vi "Add Error.vi"(8 "error in (no error)":errorcluster, 9 "String to Append":string, 10 "Error":T1, 11 "Insert Error":bool=TRUE) -> (0 "error out":errorcluster)   [LabVIEW 2021, in "Iceoryx.lvlib"]
doc: "This VI will insert a custome error message. This wrapper is designed to be inlined to minimize overhead when there is no error. It calls an error core VI that should not be inlined to minimize memory impact."
uses:
  Iceoryx.lvlib
  typedef/Errors.ctl
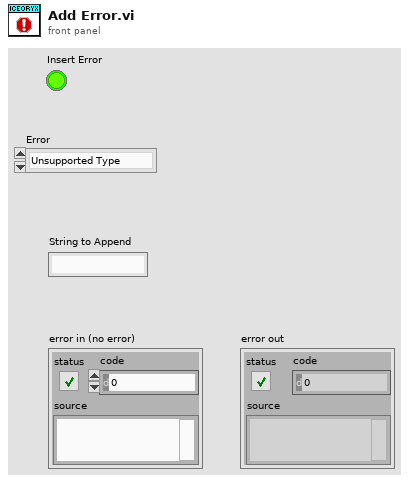
[diagram p1: front panel]
types:
  T1 = typedef "Iceoryx.lvlib/Errors.ctl" = enum16{"Unsupported Type", "Empty Name"}
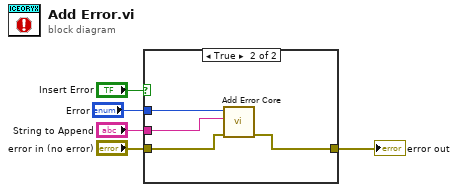
[diagram p0: block diagram]
diagram:
  n1 = case shown="True" "Insert Error" {
    tunnel: [w6 w9] -> w4
    tunnel: "error in (no error)" -> [w6 w10]
    tunnel: "Error" -> [_ w7]
    tunnel: "String to Append" -> [_ w8]
    frame False {
    }
    frame True {
      n2 = call "Add Error Core.vi"("error in (no error)"=w10, "String to Append"=w8, "Error"=w7) -> ("error out"=w9:errorcluster)  [unwired: 8 in]
    }
  }
  "error out" <- w4
